vi "Global.vi"() -> ()   [LabVIEW 2015, in "AIT 429 Shared.lvlib"]
uses:
  AIT 429 Shared.lvlib
panel:
  in  "FPGA Transmit":string="FPGA Transmit"
  in  "FPGA RT Path":string="FPGA RT Path"
  in  "Init Failed":string="Init Failed"
  in  "FPGA Type":string="FPGA Type"
  in  "FPGA Path":string="FPGA Path"
  in  "FPGA Checksum":string="FPGA Checksum"
  in  "FPGA Name":string="FPGA Name"
  in  "FPGA Reference":string="FPGA Reference"
  in  "SEA9811conf":string="SEA9811conf"
  in  "MainDisabled SEA":string="cc77431d-ab9a-4958-b642-c6ec550f90bf"
  in  "MainEnabled SEA":string="b6bddf69-436f-497a-b1b5-8a86a0639f81"
  in  "Timestamp Channel GUID (default)":string="03D3BB99-1485-13A6-561D1F898F032919"
  in  "bufferSize":string="bufferSize"
  in  "TransferType":string="TransferType"
  in  "Word Section Page GUID":string="c976e646-a24d-488b-9d95-5bd8d1727224"
  in  "Specify module by":string="Specify module by"
  in  "ScheduledSDI":string="ScheduledSDI"
  in  "xmlName":string="xmlName"
  in  "SDIValue":string="SDIValue"
  in  "SDI_Enabled":string="SDI_Enabled"
  in  "ScaleOffset":string="ScaleOffset"
  in  "ScaleFac":string="ScaleFac"
  in  "Signed?":string="Signed?"
  in  "InBufferSize":string="InBufferSize"
  in  "txRate":string="txRate"
  in  "DBHash":string="DBHash"
  in  "WinBinCache":string="Temp429BinFiles"
  in  "MainDisabled":string="C84F327B-5F00-A71A-4A47-A7C0FE0BF79D"
  in  "MainEnabled":string="6de686c8-271d-4eac-aefc-5952b5c6028a"
  in  "InputsReadRate":string="InputsReadRate"
  in  "InLoopTime":string="Inputs Loop Duration"
  in  "OutLoopTime":string="Outputs Loop Duration"
  in  "Status Section":string="Status"
  in  "Error Code":string="Error Code"
  in  "HWIn Late Count":string="Inputs Late Count"
  in  "HWOut Late Count":string="Outputs Late Count"
  in  "Static Chan GUID":string="620FF26C-B46F-A798-9FE7-99E7CBCC898B"
  in  "Default word":string="Default word"
  in  "Module#":string="Module#"
  in  "Status Section GUID":string="d47aa00e-f699-4d59-94c0-e2f1966f44aa"
  in  "Num Bits":string="Num Bits"
  in  "Channel Page GUID":string="2ea04988-eee4-4e83-9dd8-12eaea61e539"
  in  "Channel #":string="Channel #"
  in  "HWOutputs GUID":string="3512d02a-2029-43cc-b95c-a92ed63679f7"
  in  "HWInputs GUID":string="6b205014-7e01-4dc7-9fb4-ec708a1264b1"
  in  "Win File Path":string="Win File Path"
  in  "Start Bit":string="Start Bit"
  in  "RT File Path":string="RT File Path"
  in  "Type":string="Type"
  in  "Outputs":string="Outputs"
  in  "Inputs":string="Inputs"
  in  "transferPeriod":string="transferPeriod"
  in  "Label Section Page GUID":string="d344d039-fb12-41b4-81fc-ed75cdddcb8d"
  in  "Label Data Page GUID":string="e9f79bde-5caf-4b2b-afe3-0ce1e606e7c7"
  in  "Label":string="Label"
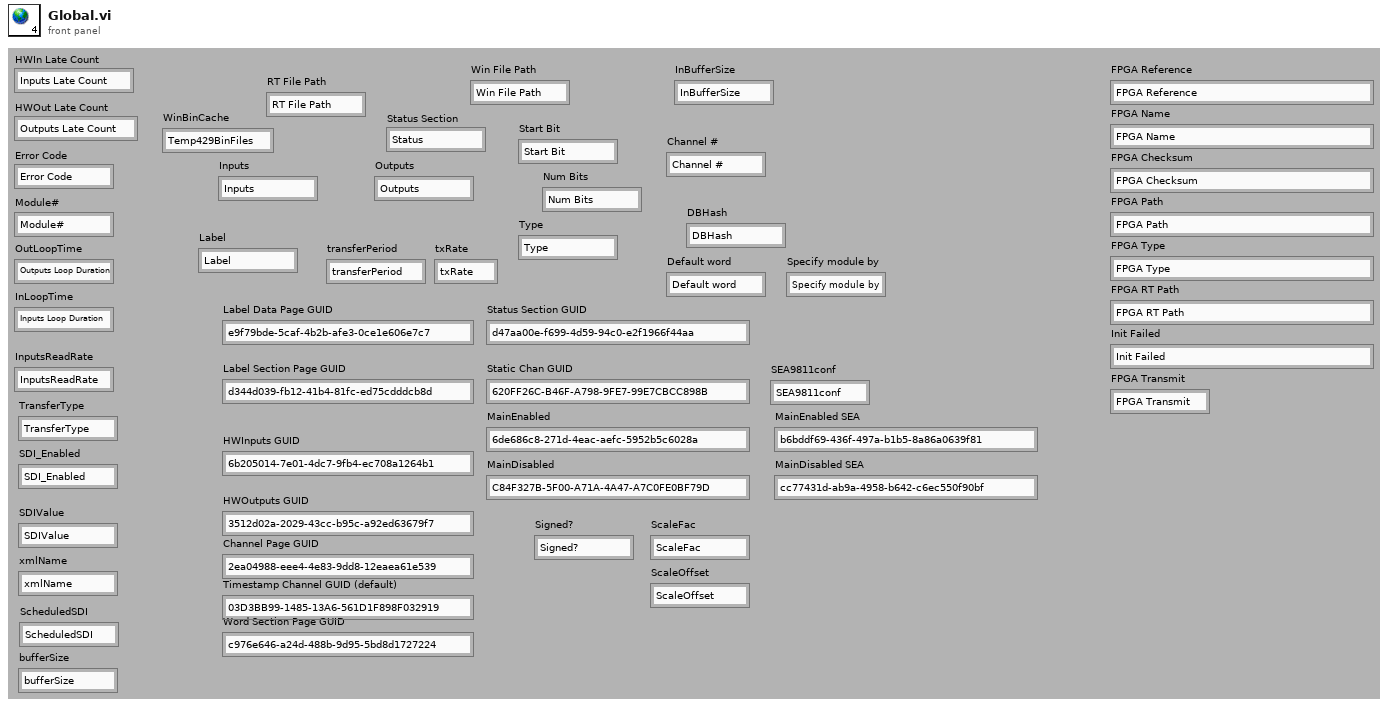
[diagram p1: front panel]
diagram:
